vi "FFT1D_CuLab.vi"(7 "Iteration":i32, 11 "samples":i32=128) -> (3 "Results(s)":dbl format="%.8f")   [LabVIEW 2020]
uses:
  9db68642-0dcb-498b-b44a-62aa3c0a4411.vi
  65ef9bab-b20b-4f39-8830-9ccf3097e1d2.vi
  <vilib>/Ngene/CuLab - GPU Accelerated Toolkit/Toolkit/Low_Level/Tensor_Classes/T_Children/T1D/T1D_Children/T1D_CSG/Pull.vi
  <vilib>/Utility/High Resolution Relative Seconds.vi
  <vilib>/Ngene/CuLab - GPU Accelerated Toolkit/Toolkit/Low_Level/GPU_Wrapper/cudart/Memory/PULL/1D/cudart_PULL_Data(CSG_1D).vi
  <vilib>/Ngene/CuLab - GPU Accelerated Toolkit/Toolkit/Low_Level/Tensor_Classes/T_Children/T1D/T1D_Children/T1D_CSG/T1D_CSG.lvclass
  C:/Program Files/National Instruments/LabVIEW 2020/vi.lib/Ngene/CuLab - GPU Accelerated Toolkit/Toolkit/Low_Level/Tensor_Classes/Tensor.lvclass
  C:/Program Files/National Instruments/LabVIEW 2020/vi.lib/Ngene/CuLab - GPU Accelerated Toolkit/Toolkit/Low_Level/Tensor_Classes/T_Children/T1D/T1D.lvclass
  <vilib>/Ngene/CuLab - GPU Accelerated Toolkit/Toolkit/Low_Level/GPU_Wrapper/cudart/cudart_get_Error_String.vi
  <vilib>/Ngene/CuLab - GPU Accelerated Toolkit/Toolkit/Low_Level/GPU_Wrapper/cudart/Memory/Utils/cudart_get_type_size(inBytes).vi
  <vilib>/Ngene/CuLab - GPU Accelerated Toolkit/Toolkit/Low_Level/Tensor_Classes/T_Children/T1D/Property/Get_Dims.vi
  <vilib>/Ngene/CuLab - GPU Accelerated Toolkit/Toolkit/Low_Level/Tensor_Classes/Property/Get_Mem_Desc.vi
  <vilib>/Ngene/CuLab - GPU Accelerated Toolkit/Toolkit/Low_Level/Checkers/Check_Tensor_Ref.vi
  <vilib>/Ngene/CuLab - GPU Accelerated Toolkit/Toolkit/API/Signal Processing/Transforms/CU_FFT/T1D/CU_FFT_T1D_C2C.vi
  <vilib>/Ngene/CuLab - GPU Accelerated Toolkit/Toolkit/Low_Level/Tensor_Classes/T_Children/T1D/T1D_Children/T1D_CSG/Push.vi
  <vilib>/Ngene/CuLab - GPU Accelerated Toolkit/Toolkit/Low_Level/Tensor_Classes/T_Children/T1D/T1D_Children/T1D_CSG/Create.vi
  <vilib>/Analysis/NI_AALBase.lvlib
  <vilib>/Ngene/CuLab - GPU Accelerated Toolkit/Toolkit/CuLab.lvlib
panel:
  out "error out":errorcluster
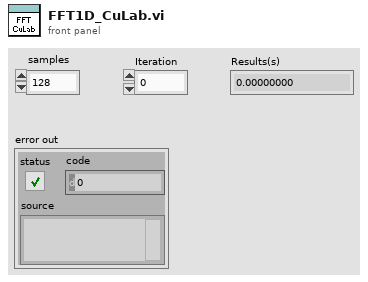
[diagram p1: front panel]
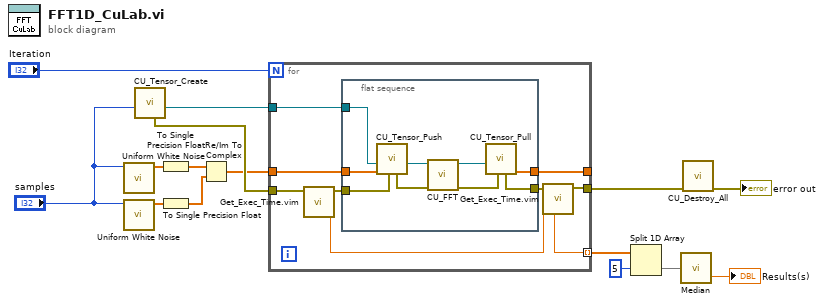
[diagram p0: block diagram]
diagram:
  n1 = call <vilib>:"Uniform White Noise.vi"("samples"="samples") -> ("uniform white noise"=w12:dbl[])  [unwired: 9 in, 1 out]
  n2 = call <vilib>:"Uniform White Noise.vi"("samples"="samples") -> ("uniform white noise"=w7:dbl[])  [unwired: 9 in, 1 out]
  n3 = call-poly <vilib>:"CU_Tensor_Create.vi"("Length"="samples") -> ("T1D_CSG out"=w13:refnum<class "T1D_CSG.lvclass">, "error out"=w10:errorcluster)  [unwired: 9 in]
  n4 = To Single Precision Float(number=w12) -> (single precision float=w11:sgl[])
  n5 = To Single Precision Float(number=w7) -> (single precision float=w6:sgl[])
  n6 = Re/Im To Complex(1:w6, 2:w11) -> (0:w5:csg[])
  n7 = for {
    N: "Iteration" -> [_]
    tunnel: w5 -> [w17]
    tunnel: w13 -> [w24]
    tunnel: w10 -> [w19]
    tunnel: [w20] -> w9
    tunnel: [w22] -> w14 mode=indexing
    tunnel: [w16] -> _
    n8 = call "Get_Exec_Time.vim"("error in (no error)"=w19) -> ("T(n)"=w23:dbl, "error out"=w18:errorcluster)  [unwired: 6 in, 1 out]
    n9 = flat-sequence {
      tunnel: w24 -> [w30]
      tunnel: [w28] -> w21
      tunnel: w18 -> [w27]
      tunnel: w17 -> [w26]
      tunnel: [w25] -> w16
      frame #0 {
        n10 = call-poly <vilib>:"CU_Tensor_Push.vi"("error in (no error)"=w27, "CPU_Data_1D_CSG"=w26, "T1D_CSG in"=w30) -> ("T1D_CSG out"=w33:refnum<class "T1D_CSG.lvclass">, "error out"=w32:errorcluster)  [unwired: 7 in]
        n11 = call-poly <vilib>:"CU_FFT.vi"("error in"=w32, "X"=w33) -> ("error out"=w31:errorcluster, "FFT {X}"=w29:refnum<class "T1D_CSG.lvclass">)  [unwired: 8 in]
        n12 = call-poly <vilib>:"CU_Tensor_Pull.vi"("error in (no error)"=w31, "T1D_CSG in"=w29) -> ("Dest out"=w25:csg[], "error out"=w28:errorcluster)  [unwired: 7 in, 1 out]
      }
    }
    n13 = call "Get_Exec_Time.vim"("T(n-1)"=w23, "error in (no error)"=w21) -> ("error out"=w20:errorcluster, "dT"=w22:dbl)  [unwired: 5 in, 1 out]
  }
  n14 = Split 1D Array(array=w14, index=5) -> (second subarray=w1:dbl[])  [unwired: 1 out]
  n15 = call <vilib>:"Median.vi"("X"=w1) -> ("median"=→"Results(s)":dbl)  [unwired: 1 out]
  n16 = call <vilib>:"CU_Destroy_All.vi"("error in"=w9) -> ("error out"=→"error out":errorcluster)  [unwired: 10 in]
